vi "Main.vi"() -> ()   [LabVIEW 2016, in "CSV Analyzer.lvlib"]
uses:
  CSV Analyzer.lvlib
  Source/SLL Table/SLL Table.lvclass
  <vilib>/Utility/error.llb/DialogType.ctl
  Source/SLL Queued State Machine/Queue Driver/Create Queue.vi
  Source/SLL Queued State Machine/Queue Driver/Enqueue an Item to Queue.vi
  Source/SLL Queued State Machine/Queue Driver/Dequeue Queue.vi
  <vilib>/Utility/file.llb/Read From Spreadsheet File (string).vi
  Source/SLL Table/_SubVIs/Get Table Data.vi
  Source/SLL Queued State Machine/Queue Driver/Enqueue N Items.vi
  Source/SLL Queued State Machine/Queue Driver/Flush Queue.vi
  Source/SLL Queued State Machine/Queue Driver/Release Queue.vi
  Source/SLL Queued State Machine/SLL QSM.lvlib
  Source/SLL File IO/Spreadsheet/SLL Spreadsheet.lvlib
panel:
  in  "Delimiter":string(combo)=","
  in  "Use LabVIEW File Read?":bool
  in  "CSV File Path":path
  out "Total Columns":i32
  out "Total Rows":i32
  in  "Headers to List[]":string[](array[combo])
  in  "Column Conditions[]":cluster{"Header":string, "Value[]":string[]}[](array[cluster])
  out "Status":string
  in  "Analyze":bool
  out "Displayed Column Count":i32
  out "Displayed Row Count":i32
  in  "Mini Table":bool
  in  "2D Data Out[][]":i32(listbox)
  # "CSV Analyzer"
  # "Empty: Displays All Columns"
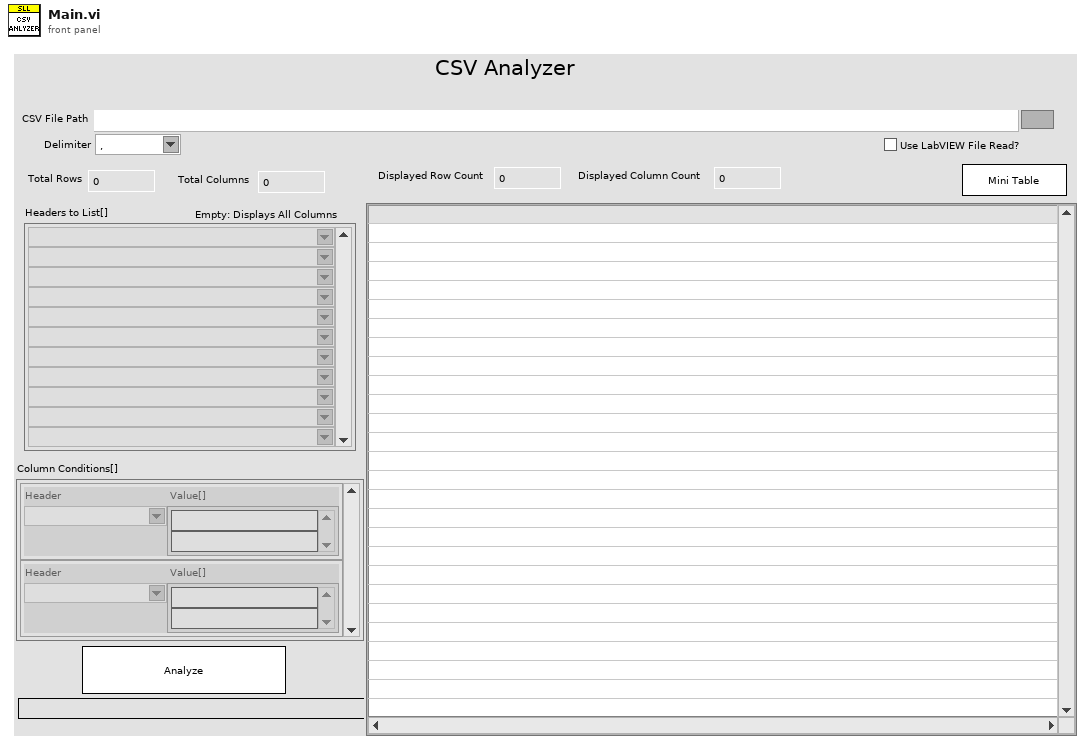
[diagram p1: front panel]
types:
  T1 = cluster{"Flags":cluster{"Source Code?":bool}, "SLL Table":refnum<class "SLL Table.lvclass">, "Headers[]":string[]}
  T2 = typedef "DialogType.ctl" = u16
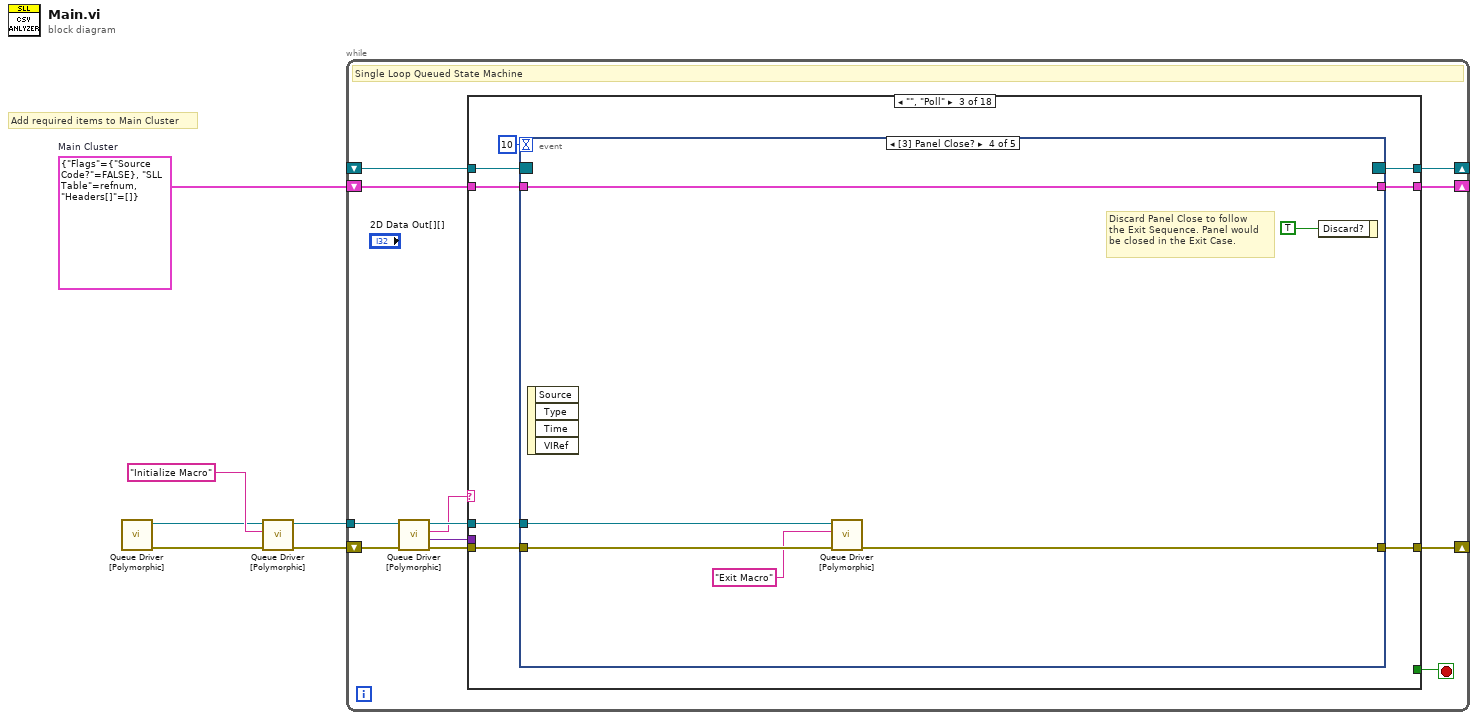
[diagram p0: block diagram]
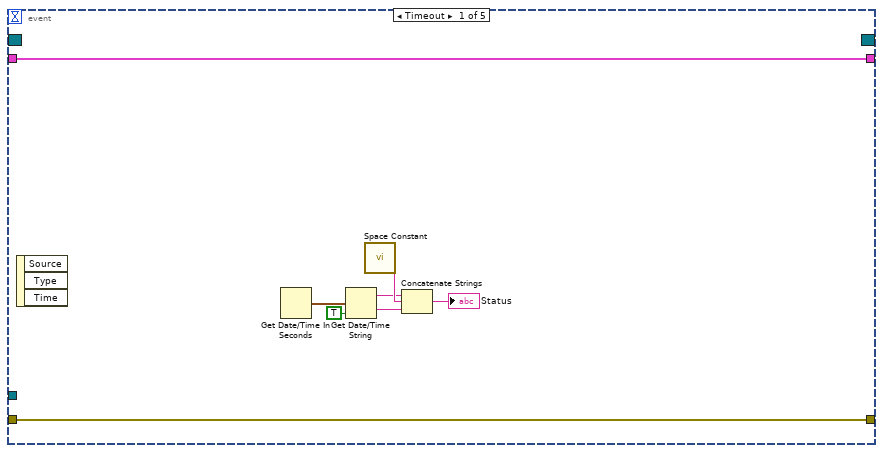
[diagram p4: hidden frame]
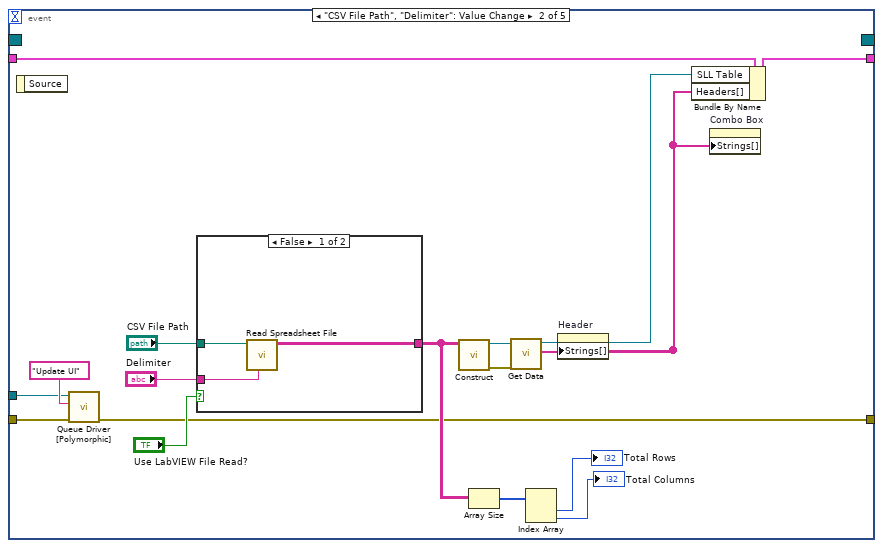
[diagram p5: hidden frame]
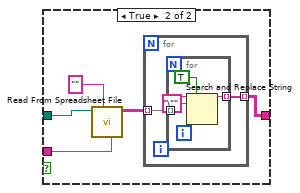
[diagram p6: hidden frame]
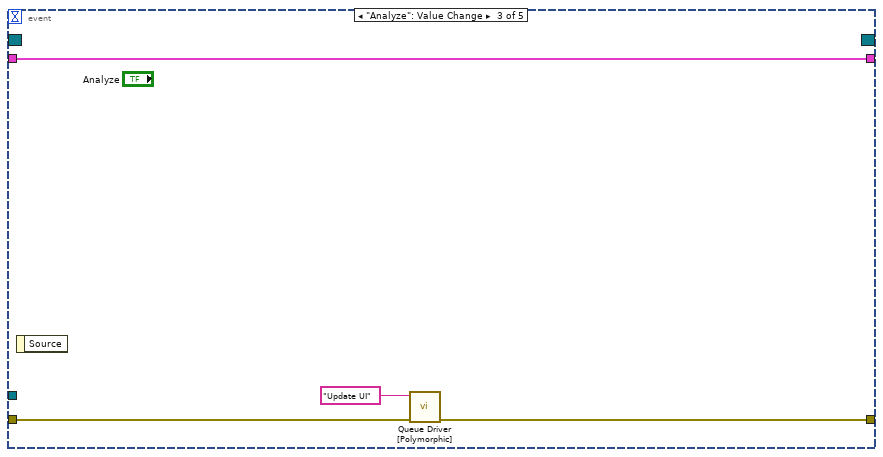
[diagram p7: hidden frame]
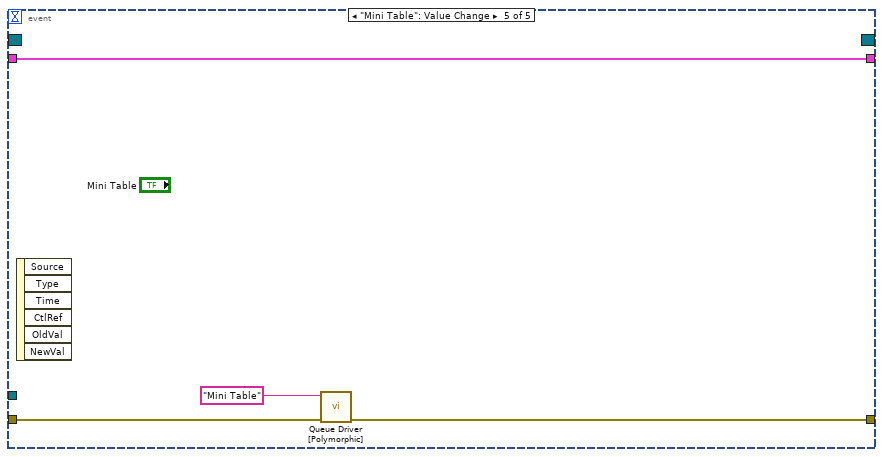
[diagram p8: hidden frame]
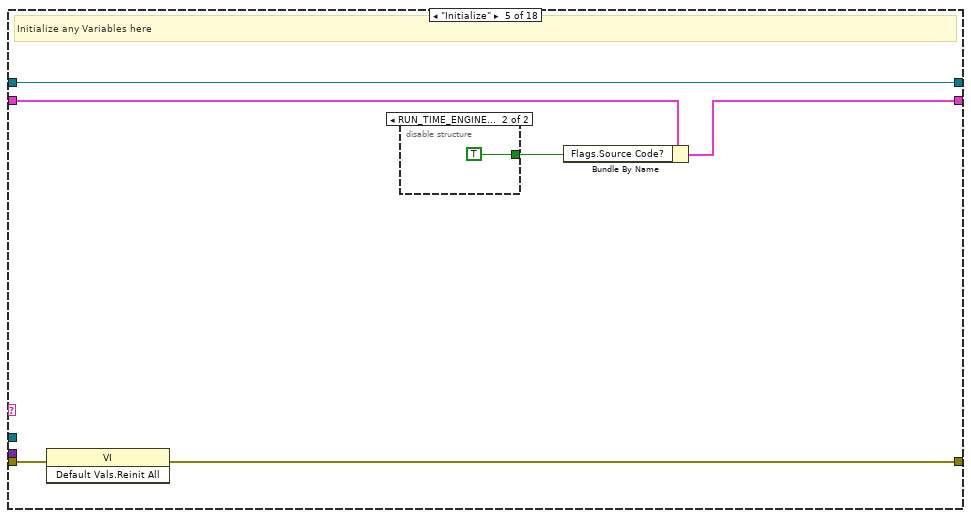
[diagram p10: hidden frame]
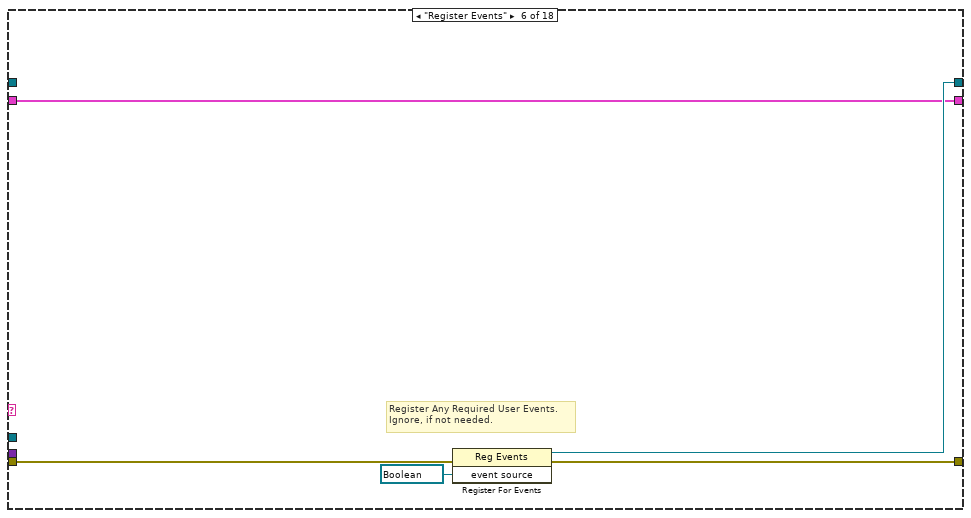
[diagram p12: hidden frame]
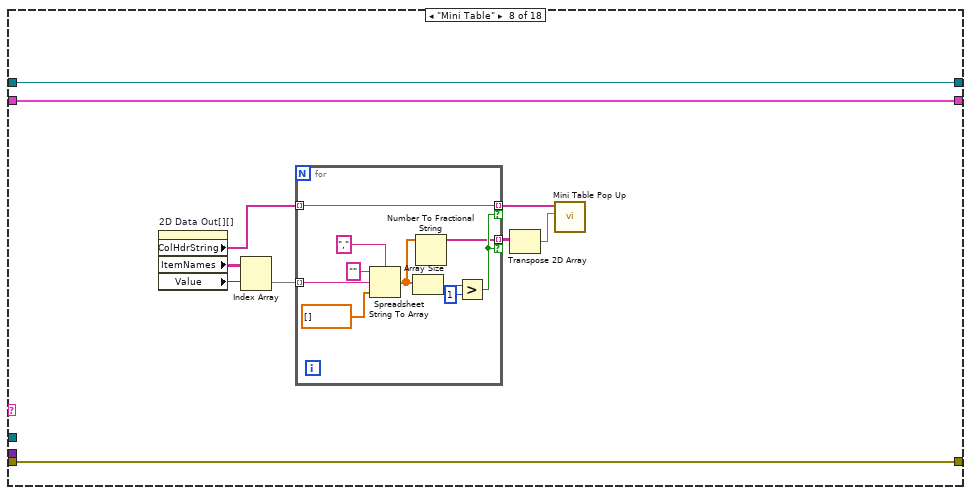
[diagram p14: hidden frame]
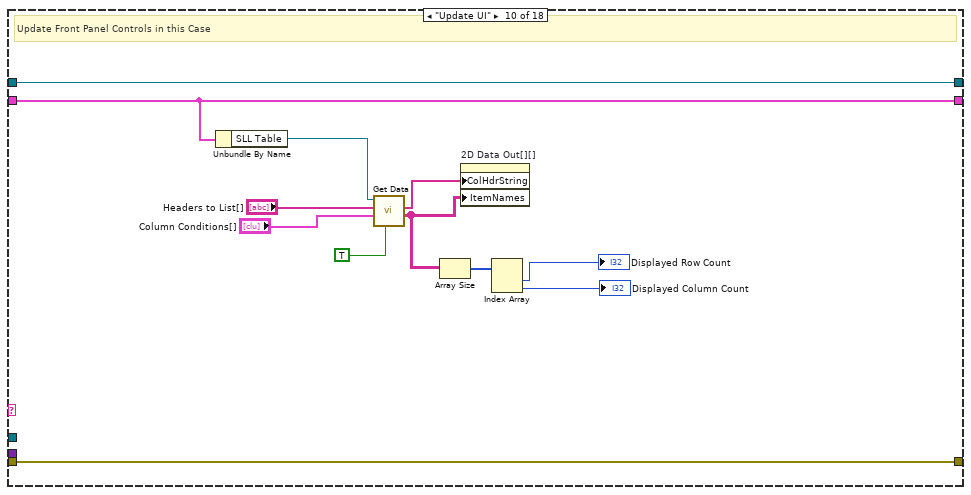
[diagram p16: hidden frame]
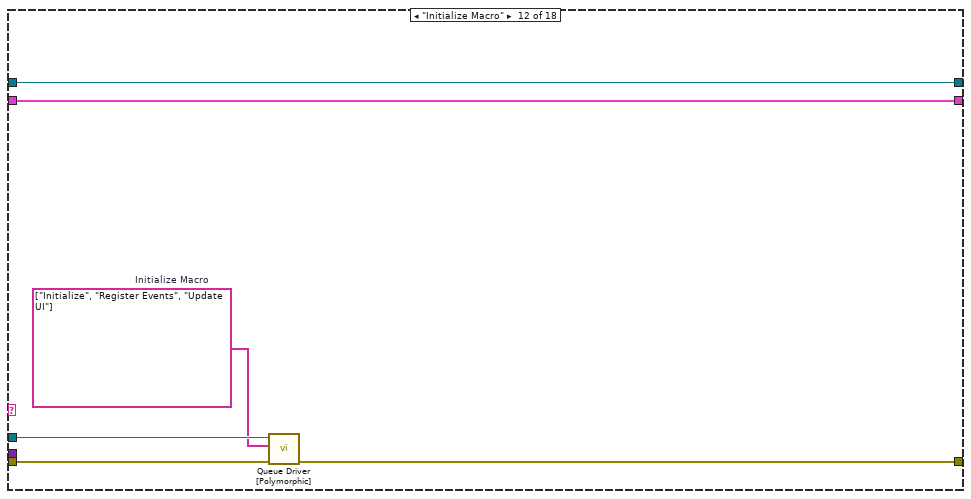
[diagram p18: hidden frame]
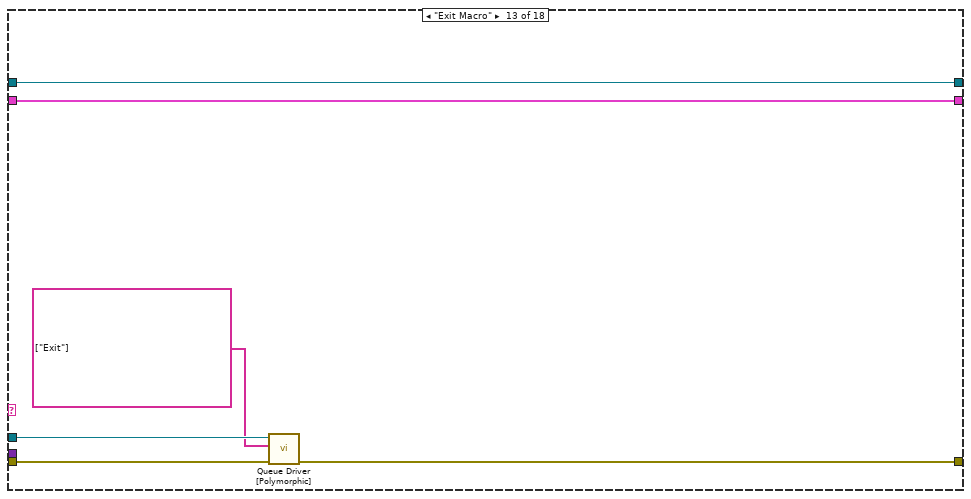
[diagram p19: hidden frame]
diagram:
  w6 = T1 {"Flags"={"Source Code?"=FALSE}, "SLL Table"=refnum, "Headers[]"=[]}  # Main Cluster
  # "Add required items to Main Cluster"
  n1 = call-poly "Queue Driver [Polymorphic].vi"() -> ("Error Out"=w5:errorcluster, "Queue Ref"=w2:refnum<queue>)  [unwired: 10 in]
  n2 = call-poly "Queue Driver [Polymorphic].vi"("Error In"=w5, "Item to Add"="Initialize Macro", "Queue Ref In"=w2) -> ("Error Out"=w4:errorcluster, "Queue Ref Out"=w1:refnum<queue>)  [unwired: 7 in]
  n3 = while "SLL Queued State Machine" {
    shift-right: [w16] -> _
    shift-left: w4 -> [w18]
    shift-right: [w13] -> _
    shift-left: _ -> [w12]
    shift-right: [w11] -> _
    shift-left: w6 -> [w10]
    tunnel: w1 -> [w8]
    stop <- w15 stop-if-true
    # "Single Loop Queued State Machine"
    n4 = call-poly "Queue Driver [Polymorphic].vi"("Error In"=w18, "Queue Ref In"=w8) -> ("Error Out"=w17:errorcluster, "Data"=w7:variant, "Dequeue"=w9:string, "Queue Ref Out"=w14:refnum<queue>)  [unwired: 6 in]
    n5 = case "QSM Case Structure" shown="\"\", \"Poll\"" w9 {
      selector: w9 -> [_ _ _ _ _ _ _ _ _ _ _ _ _ _ w157 _ _ _]
      tunnel: w17 -> [w21 w24 w30 w88 w89 w100 w103 w113 w126 w138 w141 w145 w151 w156 w160 w172 w175 w190]
      tunnel: [w21 w24 w31 w88 w90 w99 w103 w113 w126 w138 w141 w144 w150 w156 w163 w170 w175 w186] -> w16
      tunnel: [_ _ _ _ _ _ _ _ _ _ _ _ _ _ _ _ _ TRUE] -> w15
      tunnel: [w20 w23 w29 w87 w94 w98 w102 w112 w125 w137 w140 w147 w153 w155 w166 w169 w174 w189] -> w13
      tunnel: w12 -> [w20 w23 w28 w87 w94 _ w102 w112 w125 w137 w140 w147 w153 w155 w166 w169 w174 w189]
      tunnel: [w19 w22 w26 w86 w91 w97 w101 w111 w124 w128 w139 w146 w152 w154 w165 w168 w173 w188] -> w11
      tunnel: w10 -> [w19 w22 w27 w86 w92 w97 w101 w111 w124 w128 w139 w146 w152 w154 w165 w168 w173 w188]
      tunnel: w14 -> [_ _ w25 _ _ _ _ _ _ _ _ w143 w149 _ _ _ _ w177]
      tunnel: w7 -> [_ _ _ _ _ _ _ _ _ _ _ _ _ _ _ _ _ _]
      frame "/--------------- Read Me -----------------/" {
        # "General Purpose Queue Based State Machine for Any Use Case (main application, module, pop up message etc)\n\nAdvantages:\n1. No Need to Pass Queue References between Queue Driver VIs.\n2. This template can be safely used in multiple parallel running modules without any issues.\n3. This template can also be safely used even in cases where the VI is configured to be a Clone, where multiple \ninstances of the VI could be executing concurrently.\n\nHow to Use:\n1. Add necessary items to the Main Cluster.\n2. Use the Polymorphic Queue Driver for doing any queue operations. There is no need to pass the queue driver\nreference, as the Queue Driver automatically infers the reference based on the VI instance from which it is called.\n3. Add any required user events in the \"Register Events\" case. Ignore if not needed.\n4. Use \"Sequences\" section for defining any list of state calls, which could be used in multiple places. \nEg: Initialize Sequence, might be needed if we need to any reinitialization."
      }
      frame "/------------------ Poll -------------------/" {
      }
      frame "", "Poll" {
        n6 = event shown="[3] Panel Close?" {
          selector: w28 -> [_ _ _ _ _]
          dyn-events: [_ _ _ _ _] -> w29
          timeout: 10 -> [_ _ _ _ _]
          tunnel: [w40 w41 w73 w80 w84] -> w31
          tunnel: w30 -> [w40 w42 w72 w81 w85]
          tunnel: w27 -> [w39 w53 w75 w79 w83]
          tunnel: [w39 w55 w75 w79 w83] -> w26
          tunnel: w25 -> [_ w43 _ w77 _]
          event Timeout {
            n7 = event-data() -> ()  [unwired: 1 in, 3 out]
            n8 = Get Date/Time In Seconds() -> (seconds since 1Jan1904=w38:timestamp)
            n9 = Get Date/Time String(seconds (now)=w38, want seconds? (F)=TRUE) -> (date string=w34:string, time string=w33:string)  [unwired: 1 in]
            n10 = call <vilib>:"Space Constant.vi"() -> ("String"=w35:string)
            n11 = Concatenate Strings(w34, w35, w33) -> (→"Status":string)
          }
          event "CSV File Path", "Delimiter": Value Change {
            n12 = event-data() -> ()  [unwired: 1 in, 1 out]
            n13 = call-poly "Queue Driver [Polymorphic].vi"("Error In"=w42, "Item to Add"="Update UI" ("Enqueue"), "Queue Ref In"=w43) -> ("Error Out"=w41:errorcluster)  [unwired: 7 in, 1 out]
            n14 = case shown="False" "Use LabVIEW File Read?" {
              tunnel: [w60 w62] -> w51
              tunnel: "CSV File Path" -> [w59 w65]
              tunnel: "Delimiter" -> [w58 w61]
              frame False {
                n15 = call "Read Spreadsheet File.vi"("Delimiter (tab)"=w58, "File Path"=w59) -> ("2D Array"=w60:string[][])  [unwired: 8 in, 1 out]
              }
              frame True {
                n16 = call-poly <vilib>:"Read From Spreadsheet File.vi"("delimiter (\\t)"=w61, "format (%s)"="", "file path (dialog if empty)"=w65) -> ("all rows"=w63:string[][])  [unwired: 4 in, 4 out]
                n17 = for {
                  tunnel: w63 -> [w67] mode=indexing
                  tunnel: [w66] -> w62 mode=indexing
                  n18 = for {
                    tunnel: w67 -> [w71] mode=indexing
                    tunnel: [w69] -> w66 mode=indexing
                    n19 = Search and Replace String(replace all?=TRUE ("replace all? (F)"), input string=w71, search string="\"") -> (result string=w69:string)  [unwired: 5 in, 3 out]
                  }
                }
              }
            }
            n20 = call "Construct.vi"("2D String with Headers"=w51) -> ("error out"=w57:errorcluster, "Table"=w56:refnum<class "SLL Table.lvclass">)  [unwired: 9 in]
            n21 = Array Size(array=w51) -> (size(s)=w50:i32[])
            n22 = call-poly "Get Data.vi"("error in (no error)"=w57, "SLL Table in"=w56) -> ("Headers Out[]"=w45:string[], "SLL Table out"=w54:refnum<class "SLL Table.lvclass">)  [unwired: 6 in, 2 out]
            n23 = Index Array(array=w50) -> (element #1=→"Total Rows":i32, element #2=→"Total Columns":i32)  [unwired: 2 in]
            n24 = property on="Header" class="CmbBox"("Strings[]"=w45) -> ()  [unwired: 2 in, 2 out]
            n25 = Bundle By Name(cluster=w53, "SLL Table"=w54, "Headers[]"=w45) -> (w55:T1)
            n26 = property on="Combo Box" class="CmbBox"("Strings[]"=w45) -> ()  [unwired: 2 in, 2 out]
          }
          event "Analyze": Value Change {
            n27 = event-data() -> ()  [unwired: 1 in, 1 out]
            n28 = call-poly "Queue Driver [Polymorphic].vi"("Error In"=w72, "Queue Name (Optional)"="Update UI" ("Enqueue")) -> ("Error Out"=w73:errorcluster)  [unwired: 8 in, 1 out]
          }
          event Panel Close? {
            # "Discard Panel Close to follow\nthe Exit Sequence. Panel would\nbe closed in the Exit Case."
            n29 = event-data() -> ()  [unwired: 1 in, 4 out]
            n30 = call-poly "Queue Driver [Polymorphic].vi"("Error In"=w81, "Item to Add"="Exit Macro" ("Enqueue"), "Queue Ref In"=w77) -> ("Error Out"=w80:errorcluster)  [unwired: 7 in, 1 out]
            n31 = event-data("Discard?"=TRUE) -> ()  [unwired: 1 in, 1 out]
          }
          event "Mini Table": Value Change {
            n32 = event-data() -> ()  [unwired: 1 in, 6 out]
            n33 = call-poly "Queue Driver [Polymorphic].vi"("Error In"=w85, "Queue Name (Optional)"="Mini Table" ("Enqueue")) -> ("Error Out"=w84:errorcluster)  [unwired: 8 in, 1 out]
          }
        }
      }
      frame "/--------------- Initialize -----------------/" {
      }
      frame "Initialize" {
        # "Initialize any Variables here"
        n34 = invoke class="VI" method="Default Vals.Reinit All"(error in=w89) -> (error out=w90:errorcluster)  [unwired: 2 in, 2 out]
        n35 = disable-structure shown="RUN_TIME_ENGINE==False" {
          disable-tunnel: [_ TRUE] -> w93
          frame condition #0 {
          }
          frame condition #1 (active) {
          }
        }
        n36 = Bundle By Name(cluster=w92, "Flags.Source Code?"=w93) -> (w91:T1)
      }
      frame "Register Events" {
        # "Register Any Required User Events. \nIgnore, if not needed."
        n37 = register-events(error in=w100, refnum<vi> refnum ("event source")) -> (reference out=w98:refnum<event-registration>, error out=w99:errorcluster)  [unwired: 1 in]
      }
      frame "/---------- Custom Case Splitter ----------/" {
      }
      frame "Mini Table" {
        n38 = property on="2D Data Out[][]" class="MCListbox (strict)"() -> ("ColHdrString"=w107:string[], "ItemNames"=w110:string[][], "Value"=w109:i32)  [unwired: 2 in, 2 out]
        n39 = Index Array(array=w110, index (row)=w109) -> (element=w108:string[])  [unwired: 1 in]
        n40 = for {
          tunnel: w108 -> [w123] mode=indexing
          tunnel: w107 -> [w117] mode=indexing
          tunnel: [w114] -> w105 mode=indexing if=w116
          tunnel: [w117] -> w106 mode=indexing if=w116
          n41 = Spreadsheet String To Array(delimiter (Tab)=",", format string="", spreadsheet string=w123, array type (2D Dbl)=dbl[] []) -> (array=w118:dbl[])
          n42 = Array Size(array=w118) -> (size(s)=w120:i32)
          n43 = Number To Fractional String(number=w118) -> (F-format string=w114:string[])  [unwired: 3 in]
          n44 = Greater?(x=w120, y=1) -> (0:w116:bool)
        }
        n45 = Transpose 2D Array(2D array=w105) -> (transposed array=w104:string[][])
        n46 = call "Mini Table Pop Up.vi"("Data[][]"=w104, "Headers[]"=w106) -> ()  [unwired: 9 in, 1 out]
      }
      frame "/-------------- User Interface --------------/" {
        # "Duplicate this case to create additional case splitters for readability"
      }
      frame "Update UI" {
        # "Update Front Panel Controls in this Case"
        n47 = Unbundle By Name(w128) -> ("SLL Table"=w136:refnum<class "SLL Table.lvclass">)
        n48 = call-poly "Get Data.vi"("Count? (F)"=TRUE, "Column Conditions[] (Optional)"="Column Conditions[]", "Header Order[] (Optional)"="Headers to List[]", "SLL Table in"=w136) -> ("2D Data Out[][]"=w129:string[][], "Headers Out[]"=w135:string[])  [unwired: 4 in, 2 out]
        n49 = Array Size(array=w129) -> (size(s)=w134:i32[])
        n50 = property on="2D Data Out[][]" class="MCListbox (strict)"("ColHdrString"=w135, "ItemNames"=w129) -> ()  [unwired: 2 in, 2 out]
        n51 = Index Array(array=w134) -> (element #1=→"Displayed Row Count":i32, element #2=→"Displayed Column Count":i32)  [unwired: 2 in]
      }
      frame "/----------------- Macros -----------------/" {
      }
      frame "Initialize Macro" {
        w142 = string[] ["Initialize", "Register Events", "Update UI"]  # Initialize Macro
        n52 = call-poly "Queue Driver [Polymorphic].vi"("Error In"=w145, "Enqueue N"=w142, "Queue Ref In"=w143) -> ("Error Out"=w144:errorcluster)  [unwired: 7 in, 1 out]
      }
      frame "Exit Macro" {
        n53 = call-poly "Queue Driver [Polymorphic].vi"("Error In"=w151, "Enqueue N"=string[] ["Exit"], "Queue Ref In"=w149) -> ("Error Out"=w150:errorcluster)  [unwired: 7 in, 1 out]
      }
      frame "/-------------- Error Handler--------------/" {
      }
      frame Default {
        # "Undefined Case/Spelling Errors - Show Message to Developer"
        n54 = property class="VI"(error in=w160) -> (error out=w159:errorcluster, "Name"=w158:string)  [unwired: 1 in, 1 out]
        n55 = Format Into String(format string="\"%s\" in the VI - %s" ("message"), initial string="Undefined case - ", error in=w159, w157, w158) -> (resulting string=w161:string, error out=w163:errorcluster)
        n56 = One Button Dialog(message=w161) -> ()  [unwired: 1 in, 1 out]
      }
      frame "Error" {
        w167 = T2 2 items=["no dialog", "OK message", "continue or stop message", "OK message + warnings", "continue/stop + warnings"] ("type of dialog (OK msg:1)")
        # "Handle the Error"
        n57 = call <vilib>:"Simple Error Handler.vi"("type of dialog (OK msg:1)"=w167, "error in (no error)"=w172) -> ("error out"=w171:errorcluster)  [unwired: 3 in, 4 out]
        n58 = call <vilib>:"Clear Errors.vi"("error in (no error)"=w171) -> ("error out"=w170:errorcluster)  [unwired: 5 in, 1 out]
      }
      frame "/------------------- Exit --------------------/" {
      }
      frame "Exit" {
        n59 = call-poly "Queue Driver [Polymorphic].vi"("Error In"=w190, "Queue Ref In"=w177) -> ("Error Out"=w191:errorcluster, "Queue Ref Out"=w176:refnum<queue>)  [unwired: 7 in, 1 out]
        n60 = Unbundle By Name(w188) -> ("Flags.Source Code?"=w181:bool)
        n61 = call-poly "Queue Driver [Polymorphic].vi"("Error In"=w191, "Queue Ref In"=w176) -> ("Error Out"=w187:errorcluster)  [unwired: 9 in]
        n62 = Call Chain() -> (call chain=w185:string[])
        n63 = Array Size(array=w185) -> (size(s)=w184:i32)
        n64 = Equal?(x=w184, y=1) -> (x = y?=w182:bool)
        n65 = And(x=w181, y=w182) -> (x .and. y?=w180:bool)
        n66 = case "Skip Panel Close when in Source\nCode and is the top most caller" shown="True" w180 {
          tunnel: w187 -> [w194 w196]
          tunnel: [w195 w196] -> w186
          frame False {
            # "Close Panel"
            n67 = invoke class="VI" method="FP.Close"() -> (error out=w193:errorcluster)  [unwired: 3 in, 2 out]
            n68 = Merge Errors(w194, w193) -> (w195:errorcluster)
          }
          frame True {
            # "Do Not Close Panel"
          }
        }
        n69 = property on="2D Data Out[][]" class="MCListbox (strict)"("ColHdrString"=string[] [] ("Column Header Strings[]"), "ItemNames"=string[][] [] ("2D Data Out[][] 2")) -> ()  [unwired: 2 in, 2 out]
      }
    }
  }
